vi "Set Scan Rate.vi"(8 "error in":errorcluster, 10 "IP address":string, 11 "Item Ref in":T1 format="%.0x") -> (0 "error out":errorcluster, 3 "Item Ref out":T1 format="%.0x")   [LabVIEW 2024, in "SEECD System Explorer.lvlib"]
uses:
  SEECD System Explorer.lvlib
  Shared/Globals/Property Strings.vi
  Shared/SEECD Shared.lvlib
  <vilib>/NI VeriStand/Custom Device API/Custom Device API.lvlib
  <vilib>/NI VeriStand/Custom Device API/Custom Device Item Ref.ctl
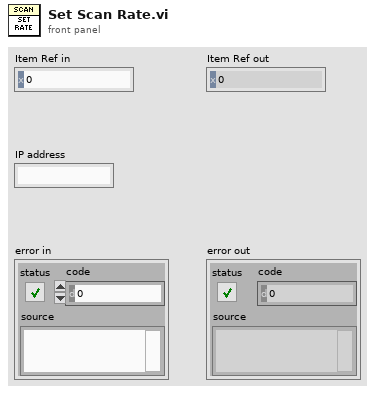
[diagram p1: front panel]
types:
  T1 = typedef "Custom Device API.lvlib/Custom Device Item Ref.ctl" = u64
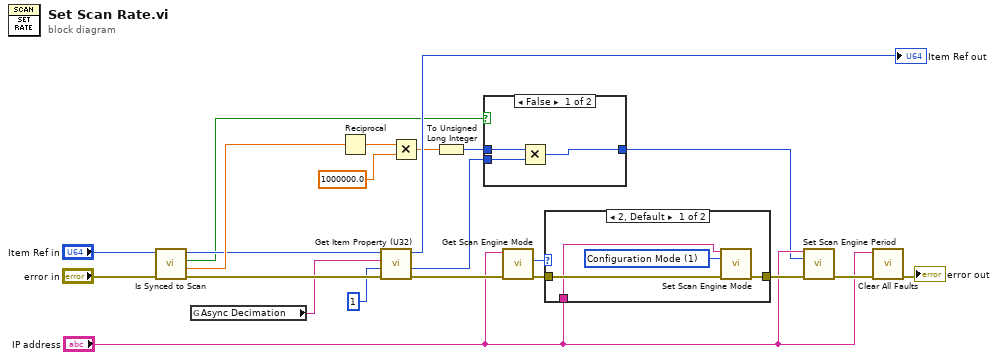
[diagram p0: block diagram]
diagram:
  n1 = call "Is Synced to Scan.vi"("error in"="error in", "Item Ref in"="Item Ref in") -> ("error out"=w19:errorcluster, "Engine Rate"=w12:dbl, "Sync to Scan?"=w6:bool, "Item Ref out"=w11:T1)  [unwired: 6 in]
  n2 = global read "Property Strings.vi" "Async Decimation"() -> (w3:string)
  n3 = Reciprocal(x=w12) -> (1/x=w9:dbl)
  n4 = call <vilib>:"Get Item Property (U32).vi"("error in (no error)"=w19, "Default Value"=u32 1, "Property Name"=w3, "Item Ref in"=w11) -> ("error out"=w21:errorcluster, "Value"=w8:u32, "Item Ref out"=→"Item Ref out":T1)  [unwired: 4 in, 1 out]
  n5 = Multiply(x=w9, y=1000000.0) -> (x*y=w4:dbl)
  n6 = To Unsigned Long Integer(number=w4) -> (unsigned 32bit integer=w10:u32)
  n7 = case shown="False" w6 {
    tunnel: w10 -> [w25 w26]
    tunnel: w8 -> [w24 _]
    tunnel: [w23 w26] -> w7
    frame False {
      n8 = Multiply(x=w25, y=w24) -> (x*y=w23:u32)
    }
    frame True {
    }
  }
  n9 = call <vilib>:"Get Scan Engine Mode.vi"("error in (no error)"=w21, "target address (localhost)"="IP address") -> ("error out"=w17:errorcluster, "mode"=w1:i32)  [unwired: 8 in]
  n10 = case shown="2, Default" w1 {
    tunnel: w17 -> [w30 w31]
    tunnel: [w29 w31] -> w16
    tunnel: "IP address" -> [w27 _]
    frame 2, Default {
      w28 = 1 items=["Configuration Mode"=1, "Active Mode"=2] ("mode (Active Mode)")
      n11 = call <vilib>:"Set Scan Engine Mode.vi"("target address (localhost)"=w27, "mode (Active Mode)"=w28, "error in (no error)"=w30) -> ("error out"=w29:errorcluster)  [unwired: 12 in]
    }
    frame 1 {
    }
  }
  n12 = call <vilib>:"Set Scan Engine Period.vi"("target address (localhost)"="IP address", "scan period (uSec)"=w7, "error in (no error)"=w16) -> ("error out"=w18:errorcluster)  [unwired: 12 in]
  n13 = call <vilib>:"Clear All Faults.vi"("error in (no error)"=w18, "target address (localhost)"="IP address") -> ("error out"=→"error out":errorcluster)  [unwired: 9 in]
